vi "UNO Q disconnect.vi"(8 "error in (no error)":errorcluster, 11 "UNO Q Session":T1={"HTTP client"=refnum, "Base URL"="", "Connected"=TRUE}) -> (0 "error out":errorcluster)   [LabVIEW 2021]
uses:
  UNO Q Session.ctl
  <vilib>/httpClient/ClientHandle.ctl
  <vilib>/httpClient/LabVIEWHTTPClient.lvlib
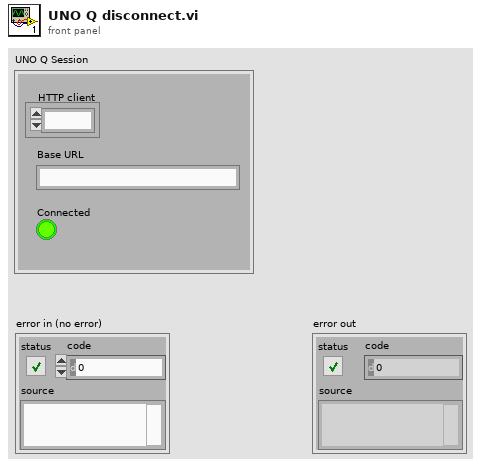
[diagram p1: front panel]
types:
  T1 = typedef "UNO Q Session.ctl" = cluster{"HTTP client":T2, "Base URL":string, "Connected":bool}
  T2 = typedef "LabVIEWHTTPClient.lvlib/ClientHandle.ctl" = refnum<k1>
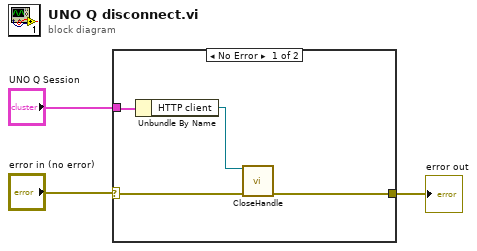
[diagram p0: block diagram]
diagram:
  n1 = case shown="No Error" "error in (no error)" {
    selector: "error in (no error)" -> [w7 w8]
    tunnel: [w6 w8] -> w2
    tunnel: "UNO Q Session" -> [w5 _]
    frame No Error {
      n2 = Unbundle By Name(w5) -> ("HTTP client"=w4:T2)
      n3 = call <vilib>:"CloseHandle.vi"("client handle"=w4, "error in (no error)"=w7) -> ("error out"=w6:errorcluster)  [unwired: 13 in]
    }
    frame Error {
    }
  }
  "error out" <- w2
